vi "Name.vi"(11 "cRIO Power Status EStop in":refnum<class "cRIO Power Status EStop.lvclass">) -> (2 "Name":string)   [LabVIEW 2025, in "VolatusControl.lvlib" / "cRIO Power Status EStop.lvclass"]
uses:
  cRIO Power Status EStop.lvclass
  cRIO Power Status EStop.lvclass/cRIO Power Status EStop.ctl
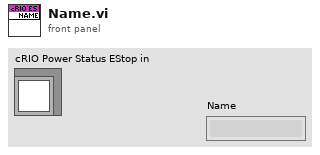
[diagram p1: front panel]
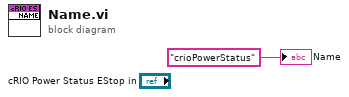
[diagram p0: block diagram]
diagram:
  "Name" <- "crioPowerStatus" ("Name")
